vi "Model--Set Value.vi"(8 "error in":errorcluster, 10 "Value":i32, 11 "Selector in":refnum<class "Selector.lvclass">) -> (0 "error out":errorcluster, 2 "element":T1, 3 "Selector out":refnum<class "Selector.lvclass">)   [LabVIEW 2019, in "Selector.lvclass"]
uses:
  Selector.lvclass
  Selector.lvclass/Selector.ctl
  Item.ctl
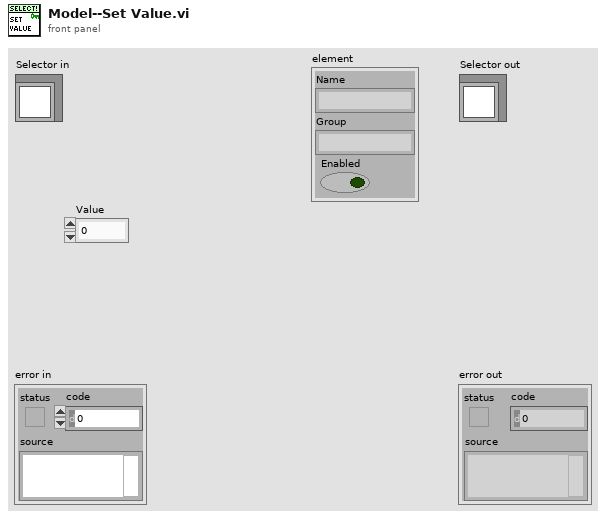
[diagram p1: front panel]
types:
  T1 = typedef "Selector.lvclass/Item.ctl" = cluster{"Name":string, "Group":string, "Enabled":bool}
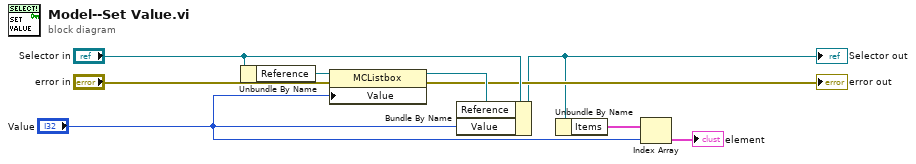
[diagram p0: block diagram]
diagram:
  n1 = Unbundle By Name("Selector in") -> ("Reference"=w9:refnum<vi>)
  n2 = property class="MCListbox"(reference=w9, error in="error in", "Value"="Value") -> (reference out=w7:refnum<vi>, error out=→"error out":errorcluster)
  n3 = Bundle By Name(cluster="Selector in", "Reference"=w7, "Value"="Value") -> (w4:refnum<class "Selector.lvclass">)
  "Selector out" <- w4
  n4 = Unbundle By Name(w4) -> ("Items"=w3:T1[])
  n5 = Index Array(array=w3, index="Value") -> (element=→"element":T1)
